vi "Launch Configurator.vi"(8 "error in (no error)":errorcluster) -> (0 "error out":errorcluster)   [LabVIEW 2021, in "Channel.lvlib"]
uses:
  Channel.lvlib
  Channel/ChannelManagerUI/ChannelManagerUI.lvclass
  C:/Program Files/National Instruments/LabVIEW 2021/vi.lib/ActorFramework/Actor/Actor.lvclass
  <vilib>/ActorFramework/Actor/Actor.lvclass
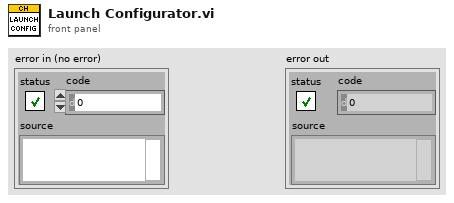
[diagram p1: front panel]
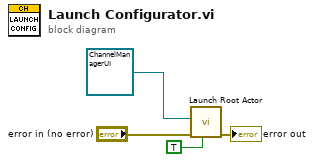
[diagram p0: block diagram]
diagram:
  n1 = call <vilib>:"Launch Root Actor.vi"("Open Actor Core front panel? (F)"=TRUE, "error in (no error)"="error in (no error)", "Actor"=refnum<class "ChannelManagerUI.lvclass"> refnum ("Channel.lvlib:ChannelManagerUI.lvlib:ChannelManagerUI")) -> ("error out"=→"error out":errorcluster)  [unwired: 7 in, 1 out]
